vi "Benchmark_TCP Connection.vi"() -> ()   [LabVIEW 2013]
uses:
  MQTT-Connection/source/MQTT_Connection/Connection/Connection.lvclass
  <vilib>/LabVIEW Open Source Project/MQTT Connection/MQTT_Base/Base Class/MQTT_Base.lvclass
  <vilib>/LabVIEW Open Source Project/MQTT TCP Connection/MQTT_TCP/Connection/TCPConnection.lvclass
panel:
  in  "with Process":bool
  out "error out":errorcluster
  out "Waveform Chart":cluster{"elapsed (s)":dbl, "elapsed (s)":dbl}(graph)
  in  "stop":bool
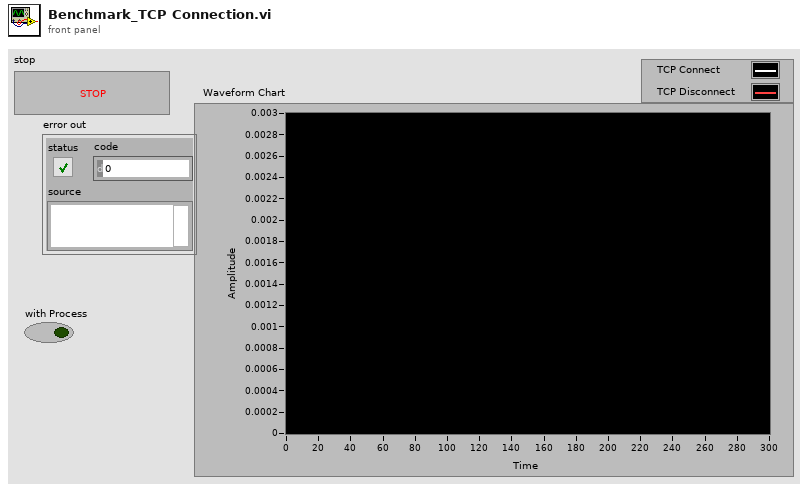
[diagram p1: front panel]
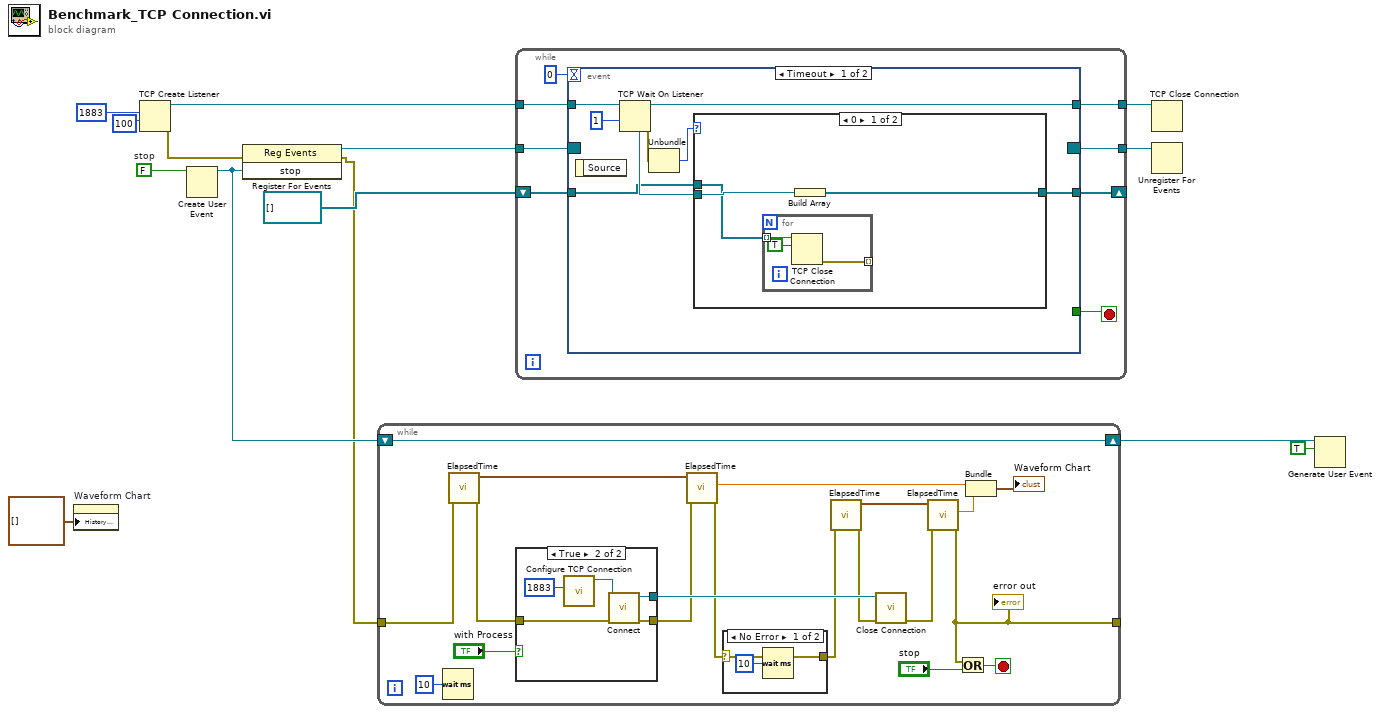
[diagram p0: block diagram]
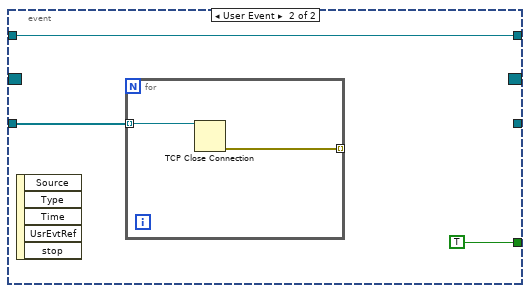
[diagram p3: hidden frame]
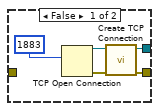
[diagram p4: hidden frame]
diagram:
  w13 = FALSE  # stop
  n1 = property on="Waveform Chart" class="WFChart (strict)"("History Data"=cluster{"elapsed (s)":dbl, "elapsed (s)":dbl}[] []) -> ()  [unwired: 2 in, 2 out]
  n2 = TCP Create Listener(9:100, 10:u16 1883 ("port")) -> (0:w1:errorcluster, 3:w5:refnum<k5>)  [unwired: 3 in, 1 out]
  n3 = Create User Event(user event datatype=w13) -> (user event=w10:refnum<user-event>)  [unwired: 1 in, 1 out]
  n4 = register-events(error in=w1, w10) -> (reference out=w9:refnum<event-registration>, error out=w2:errorcluster)  [unwired: 1 in]
  n5 = while {
    tunnel: w2 -> [w32]
    tunnel: [w15] -> _
    shift-right: [w26] -> w12
    shift-left: w10 -> [w26]
    stop <- w30 stop-if-true
    n6 = Wait (ms)(milliseconds to wait=u32 10) -> ()  [unwired: 1 out]
    n7 = call "ElapsedTime.vi"("error in"=w32) -> ("error out"=w31:errorcluster, "current time"=w24:timestamp)  [unwired: 8 in, 1 out]
    n8 = case shown="True" "with Process" {
      tunnel: [w38 w43] -> w33
      tunnel: w31 -> [_ w42]
      tunnel: [w37 w41] -> w22
      frame False {
        n9 = TCP Open Connection(remote port or service name=u16 1883) -> (connection ID=w35:refnum<k5>, error out=w36:errorcluster)  [unwired: 4 in]
        n10 = call "Create TCP Connection.vi"("error in (no error)"=w36, "connection ID"=w35) -> ("error out"=w37:errorcluster, "TCPConnection out"=w38:refnum<class "TCPConnection.lvclass">)  [unwired: 8 in]
      }
      frame True {
        n11 = call "Configure TCP Connection.vi"("remote port (80)"=u16 1883) -> ("TCPConnection"=w40:refnum<class "TCPConnection.lvclass">)  [unwired: 9 in, 1 out]
        n12 = call "Connect.vi"("error in (no error)"=w42, "Connection in"=w40) -> ("error out"=w41:errorcluster, "Connection out"=w43:refnum<class "TCPConnection.lvclass">)  [unwired: 8 in]
      }
    }
    n13 = call "ElapsedTime.vi"("error in"=w22, "compare time"=w24) -> ("error out"=w21:errorcluster, "elapsed (s)"=w23:dbl)  [unwired: 7 in, 1 out]
    n14 = case shown="No Error" w21 {
      selector: w21 -> [w44 w46]
      tunnel: [w44 w46] -> w19
      frame No Error {
        n15 = Wait (ms)(milliseconds to wait=u32 10) -> ()  [unwired: 1 out]
      }
      frame Error {
      }
    }
    n16 = call "ElapsedTime.vi"("error in"=w19) -> ("error out"=w18:errorcluster, "current time"=w20:timestamp)  [unwired: 8 in, 1 out]
    n17 = call "Close Connection.vi"("error in (no error)"=w18, "Connection in"=w33) -> ("error out"=w16:errorcluster)  [unwired: 8 in, 1 out]
    n18 = call "ElapsedTime.vi"("error in"=w16, "compare time"=w20) -> ("error out"=w15:errorcluster, "elapsed (s)"=w17:dbl)  [unwired: 7 in, 1 out]
    "error out" <- w15
    n19 = Or(x=w15, y="stop") -> (x .or. y?=w30:bool)
    n20 = Bundle("elapsed (s)"=w23, "elapsed (s)"=w17) -> (→"Waveform Chart":cluster{"elapsed (s)":dbl, "elapsed (s)":dbl})  [unwired: 1 in]
  }
  n21 = while {
    tunnel: w9 -> [w54]
    tunnel: [w53] -> w8
    tunnel: w5 -> [w51]
    tunnel: [w49] -> w4
    shift-right: [w48] -> _
    shift-left: refnum<k5>[] [] -> [w47]
    stop <- w50 stop-if-true
    n22 = event shown="[0] Timeout" {
      selector: w54 -> [_ _]
      dyn-events: [_ _] -> w53
      timeout: 0 -> [_ _]
      tunnel: w51 -> [w61 w71]
      tunnel: [_ TRUE] -> w50
      tunnel: [w59 w71] -> w49
      tunnel: [w58 _] -> w48
      tunnel: w47 -> [w57 w70]
      event Timeout {
        n23 = event-data() -> ()  [unwired: 1 in, 1 out]
        n24 = TCP Wait On Listener(9:1, 11:w61) -> (0:w56:errorcluster, 3:w59:refnum<k5>, 4:w60:refnum<k5>)  [unwired: 2 in, 2 out]
        n25 = Unbundle(w56) -> ("code"=w55:i32)  [unwired: 2 out]
        n26 = case shown="0" w55 {
          tunnel: w60 -> [w64 _]
          tunnel: [w65 w69] -> w58
          tunnel: w57 -> [w63 w69]
          frame 0 {
            n27 = for {
              tunnel: w63 -> [w68] mode=indexing
              tunnel: [w67] -> _ mode=indexing
              n28 = TCP Close Connection(connection ID=w68, abort (F)=TRUE) -> (error out=w67:errorcluster)  [unwired: 1 in, 1 out]
            }
            n29 = Build Array(w64) -> (w65:refnum<k5>[])
          }
          frame Default {
          }
        }
      }
      event User Event {
        n30 = event-data() -> ()  [unwired: 1 in, 5 out]
        n31 = for {
          tunnel: w70 -> [w74] mode=indexing
          tunnel: [w73] -> _ mode=indexing
          n32 = TCP Close Connection(connection ID=w74) -> (error out=w73:errorcluster)  [unwired: 2 in, 1 out]
        }
      }
    }
  }
  n33 = TCP Close Connection(connection ID=w4) -> ()  [unwired: 2 in, 2 out]
  n34 = Unregister For Events(event registration refnum=w8) -> ()  [unwired: 1 in, 1 out]
  n35 = Generate User Event(user event=w12, event data cluster=TRUE ("event data")) -> ()  [unwired: 2 in, 2 out]
